vi "rade-japc-test01.vi"() -> ()   [LabVIEW 2024]
uses:
  <userlib>/_RADE/cmw/server/controls/PropertySettings.ctl
  <userlib>/_RADE/cmw/server/private/CMWSSubscribe.vi
  <userlib>/_RADE/cmw/server/CMWServer.lvclass
panel:
  out "test_property":T1
  in  "error in (no error)":errorcluster
  in  "stop":bool
  out "error out":errorcluster
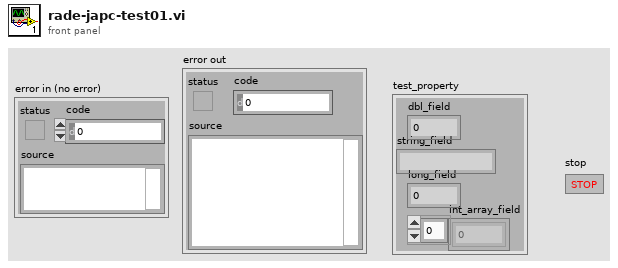
[diagram p1: front panel]
types:
  T1 = cluster{"dbl_field":dbl, "string_field":string, "long_field":i64, "int_array_field":i32[]}
  T2 = typedef "CMWServer.lvclass/PropertySettings.ctl" = cluster{"Restriction (BOTH)":enum16{"Set ONLY", "Get ONLY", "BOTH"}, "Get Type (DIRECT)":enum16{"DIRECT", "SERVERACTION"}, "Set Type (DIRECT)":enum16{"DIRECT", "SERVERACTION"}, "Persistency":bool}
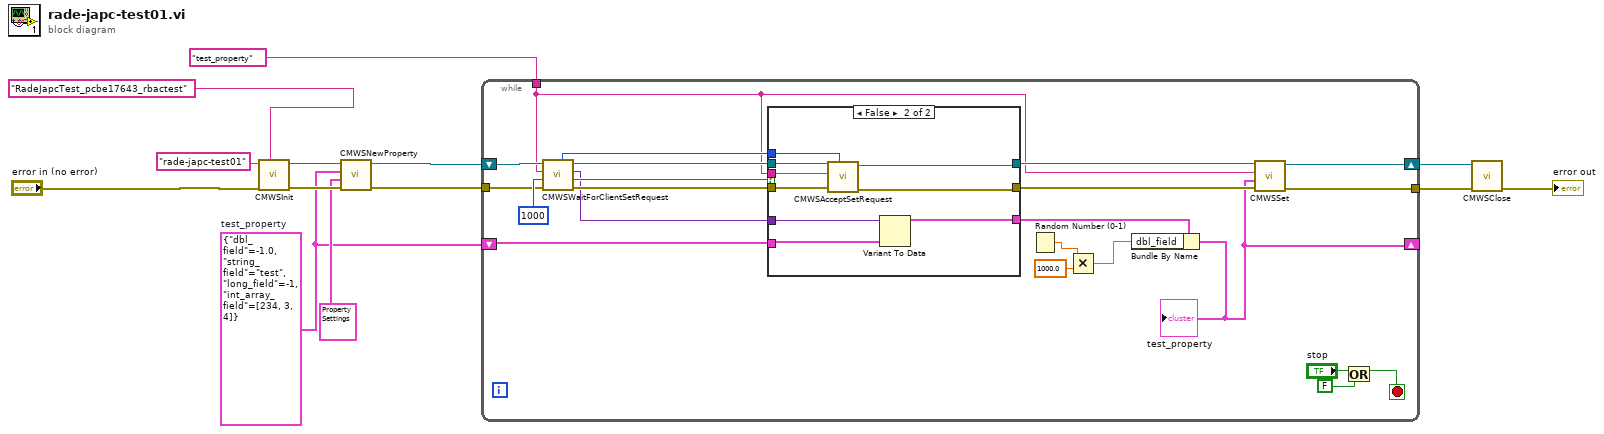
[diagram p0: block diagram]
diagram:
  w4 = T1 {"dbl_field"=-1.0, "string_field"="test", "long_field"=-1, "int_array_field"=[234, 3, 4]}  # test_property
  n1 = call <userlib>:"CMWSInit.vi"("Server Name"="RadeJapcTest_pcbe17643_rbactest", "error in (no error)"="error in (no error)", "Device Name"="rade-japc-test01") -> ("error out"=w10:errorcluster, "CMWServer"=w12:refnum<class "CMWServer.lvclass">)  [unwired: 7 in]
  n2 = call <userlib>:"CMWSNewProperty.vi"("error in"=w10, "PropertySettings"=T2 {"Restriction (BOTH)"=enum."BOTH", "Get Type (DIRECT)"=enum."DIRECT", "Set Type (DIRECT)"=enum."DIRECT", "Persistency"=FALSE}, "CMW Supported Data Type"=w4, "CMWServer in"=w12) -> ("error out"=w2:errorcluster, "CMWServer out"=w3:refnum<class "CMWServer.lvclass">)  [unwired: 6 in]
  n3 = while {
    shift-right: [w35] -> w11
    shift-left: w3 -> [w31]
    tunnel: "test_property" ("propertyName") -> [w21]
    shift-right: [w20] -> _
    shift-left: w4 -> [w23]
    tunnel: [w17] -> w8
    tunnel: w2 -> [w16]
    stop <- w18 stop-if-true
    n4 = call <userlib>:"CMWSWaitForClientSetRequest.vi"("error in"=w16, "timeout (1200)"=1000, "propertyName"=w21, "CMWServer in"=w31) -> ("error out"=w28:errorcluster, "timeout?"=w27:bool, "variant"=w24:variant, "CMWServer out"=w30:refnum<class "CMWServer.lvclass">, "requestId"=w29:i64)  [unwired: 2 in, 1 out]
    n5 = case shown="False" w27 {
      tunnel: w30 -> [w37 w47]
      tunnel: w29 -> [_ w46]
      tunnel: w28 -> [w38 w45]
      tunnel: w21 -> [_ w44]
      tunnel: [w38 w42] -> w25
      tunnel: [w37 w43] -> w26
      tunnel: w24 -> [_ w41]
      tunnel: w23 -> [w36 w40]
      tunnel: [w36 w39] -> w22
      frame True {
      }
      frame False {
        n6 = call <userlib>:"CMWSAcceptSetRequest.vi"("requestId"=w46, "error in (no error)"=w45, "propertyName"=w44, "CMWServer"=w47) -> ("error out"=w42:errorcluster, "CMWServer out"=w43:refnum<class "CMWServer.lvclass">)  [unwired: 6 in]
        n7 = Variant To Data(type=w40, Variant=w41) -> (data=w39:T1)  [unwired: 1 in, 1 out]
      }
    }
    n8 = Random Number (0-1)() -> (number: 0 to 1=w34:dbl)
    n9 = Multiply(x=w34, y=1000.0) -> (x*y=w15:dbl)
    n10 = Bundle By Name(cluster=w22, "dbl_field"=w15) -> (w20:T1)
    "test_property" <- w20
    n11 = call <userlib>:"CMWSSet.vi"("error in"=w25, "CMW Supported Data Type"=w20, "propertyName"=w21, "CMWServer"=w26) -> ("error out"=w17:errorcluster, "CMWServer out"=w35:refnum<class "CMWServer.lvclass">)  [unwired: 6 in]
    n12 = Or(x="stop", y=FALSE) -> (x .or. y?=w18:bool)
  }
  n13 = call <userlib>:"CMWSClose.vi"("error in"=w8, "CMWServer"=w11) -> ("error out"=→"error out":errorcluster)  [unwired: 9 in]
